vi "Read String.vi"(8 "error in (no error)":errorcluster, 9 "Timeout (ms)":i32, 11 "CIFTag in":refnum<class "CIF_Iceoryx_Chn_String.lvclass">) -> (0 "error out":errorcluster, 1 "timed out?":bool, 2 "Data":string, 3 "CIFTag out":refnum<class "CIF_Iceoryx_Chn_String.lvclass">)   [LabVIEW 2021, in "CIF_Iceoryx_Chn_String.lvclass"]
uses:
  CIF_Iceoryx_Chn_String.lvclass
  CIF_Iceoryx_Chn_String.lvclass/CIF_Iceoryx_Chn_String.ctl
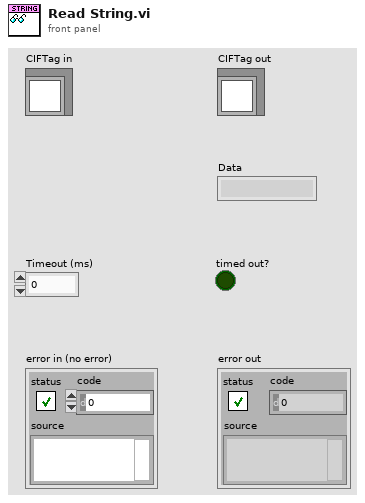
[diagram p1: front panel]
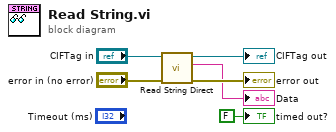
[diagram p0: block diagram]
diagram:
  n1 = call "Read String Direct.vi"("error in (no error)"="error in (no error)", "CIFTag in"="CIFTag in") -> ("error out"=→"error out":errorcluster, "Data"=→"Data":string, "CIFTag out"=→"CIFTag out":refnum<class "CIF_Iceoryx_Chn_String.lvclass">)  [unwired: 7 in]
  "timed out?" <- FALSE ("timed out?")
